vi "start daemon.vi"(8 "error in (no error)":errorcluster, 11 "context out (no context)":refnum<class "zmq_context.lvclass">) -> (0 "error out":errorcluster)   [LabVIEW 2020, in "ui-testing.lvlib"]
doc: "Start the LabVIEW UI testing daemon.\nIf you use ZeroMQ in your application make sure to <b>wire the context</b> to that VI. LabVIEW might crash otherwise or give you errors."
uses:
  ui-testing.lvlib
  <vilib>/addons/zeromq/zmq_context.lvclass
  main.vi
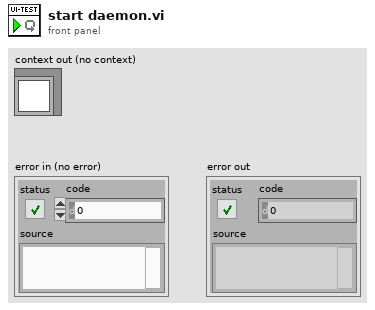
[diagram p1: front panel]
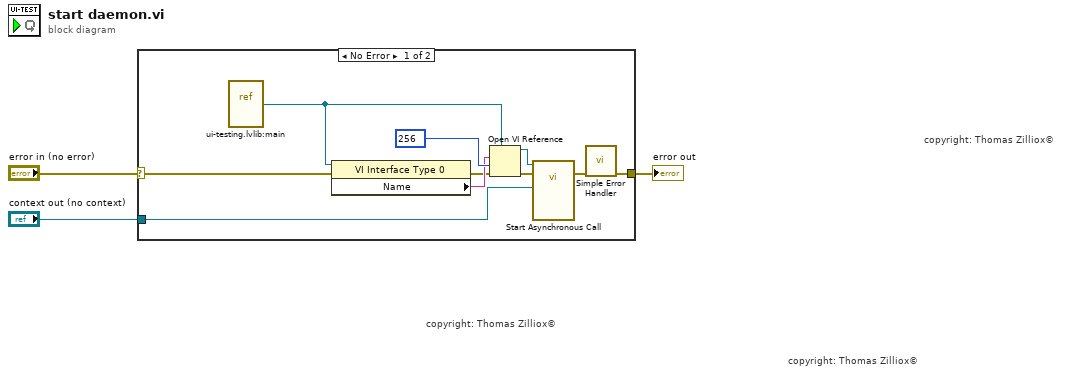
[diagram p0: block diagram]
diagram:
  # "copyright: Thomas Zilliox©"
  # "copyright: Thomas Zilliox©"
  # "copyright: Thomas Zilliox©"
  n1 = case shown="No Error" "error in (no error)" {
    selector: "error in (no error)" -> [w7 w14]
    tunnel: [w6 w14] -> w2
    tunnel: "context out (no context)" -> [w4 _]
    frame No Error {
      n2 = vi-ref "ui-testing.lvlib:main.vi"() -> (w5:refnum<vi>)
      n3 = property class="VI Interface Type 0"(reference=w5, error in=w7) -> (error out=w8:errorcluster, "Name"=w9:string)  [unwired: 1 out]
      n4 = Open VI Reference(type specifier VI Refnum (for type only)=w5, vi path=w9, options=256 ("call and forget"), error in (no error)=w8) -> (vi reference=w12:refnum<vi>, error out=w11:errorcluster)  [unwired: 2 in]
      n5 = call-by-ref "Start Asynchronous Call"(reference=w12, error in=w11, "context out"=w4) -> (error out=w10:errorcluster)  [unwired: 10 in, 2 out]
      n6 = call <vilib>:"Simple Error Handler.vi"("error in (no error)"=w10) -> ("error out"=w6:errorcluster)  [unwired: 4 in, 4 out]
    }
    frame Error {
    }
  }
  "error out" <- w2
